vi "Bridge_Process_ACK.vi"(8 "error in (no error)":errorcluster={"status"=FALSE, "code"=0, "source"="\"\""}, 10 "controller ACK":string, 11 "Dispatch ticket":string) -> (0 "error out":errorcluster={"status"=FALSE, "code"=0, "source"="\"\""}, 2 "status ok":bool, 3 "CommandStatus event":string)   [LabVIEW 2026]
doc: "INTENT: Distinguish accept/applied/achieved. LOGIC: Correlate accepted, controller applied acknowledgement and independent feedback achieved evaluation."
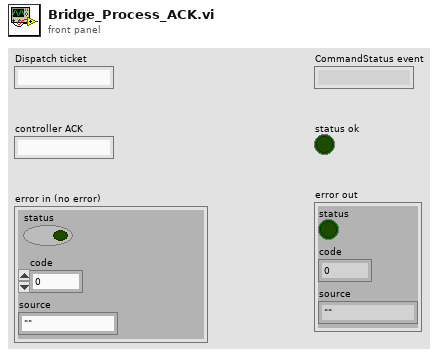
[diagram p1: front panel]
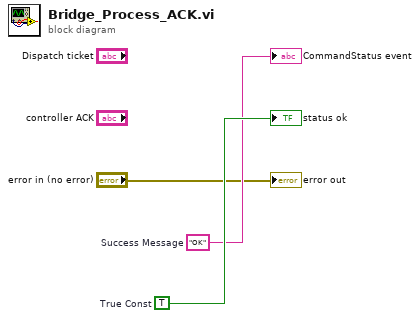
[diagram p0: block diagram]
diagram:
  w3 = TRUE  # True Const
  w2 = "OK"  # Success Message
  "CommandStatus event" <- w2
  "status ok" <- w3
  "error out" <- "error in (no error)"
